vi "getCharactersv2.vi"(0 "ocr in":refnum<class "ocr.lvclass">, 5 "noofImgs":i32=1, 11 "error in (no error)":errorcluster) -> (4 "ocr out":refnum<class "ocr.lvclass">, 6 "succ":i32, 8 "OCRResultB":T1[](array[typedef]), 15 "error out":errorcluster)   [LabVIEW 2025, in "adsOCR.lvlib" / "ocr.lvclass"]
uses:
  ocr.lvclass
  ocrImageResult.ctl
  ocrDetection.ctl
  ocr.lvclass/ocr.ctl
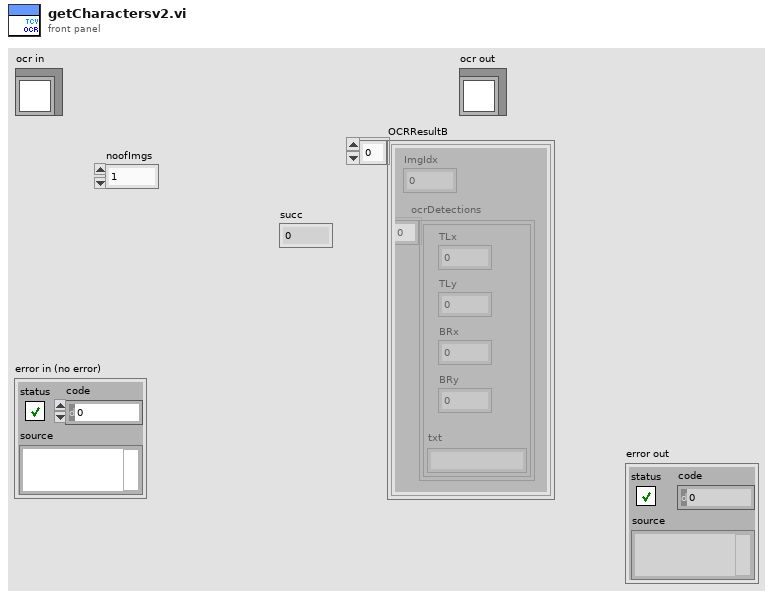
[diagram p1: front panel]
types:
  T1 = typedef "adsOCR.lvlib/ocr.lvclass/ocrImageResult.ctl" = cluster{"ImgIdx":i16, "ocrDetections":T2[]}
  T2 = typedef "adsOCR.lvlib/ocr.lvclass/ocrDetection.ctl" = cluster{"TLx":i32, "TLy":i32, "BRx":i32, "BRy":i32, "txt":string}
  T3 = typedef "adsOCR.lvlib/ocr.lvclass/TextDecRecResult2L.ctl" = cluster{"imgIdx":i32, "TLx":i32, "TLy":i32, "BRx":i32, "BRy":i32, "angle":sgl, "txtLen":i32}
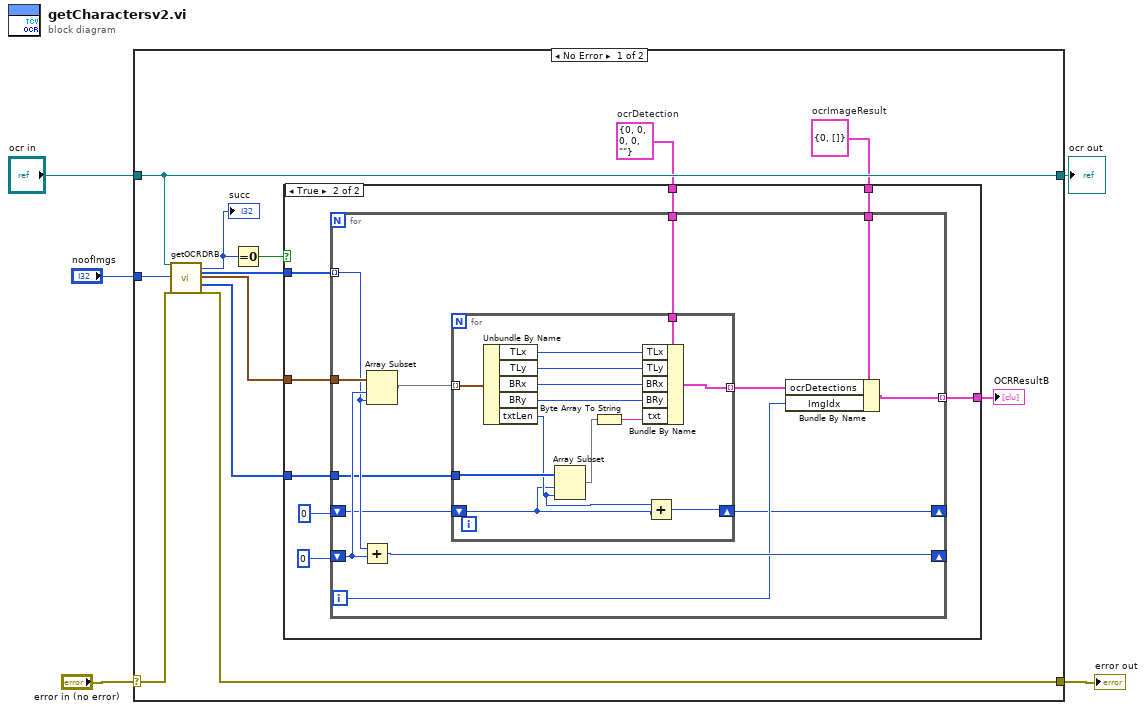
[diagram p0: block diagram]
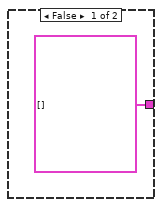
[diagram p2: hidden frame]
diagram:
  n1 = case shown="No Error" "error in (no error)" {
    selector: "error in (no error)" -> [w7 w54]
    tunnel: [w6 w54] -> w4
    tunnel: [w17 w53] -> w2
    tunnel: "ocr in" -> [w17 w53]
    tunnel: "noofImgs" -> [w16 _]
    frame No Error {
      w11 = T2 {"TLx"=0, "TLy"=0, "BRx"=0, "BRy"=0, "txt"=""}  # ocrDetection
      w9 = T1 {"ImgIdx"=0, "ocrDetections"=[]}  # ocrImageResult
      n2 = call-dynamic "getOCRDRB.vi"("ocr in"=w17, "noofImgs"=w16, "error in (no error)"=w7) -> ("succ"=w14:i32, "countsPerImg"=w13:i32[], "TextDecRecResult2L"=w12:T3[], "Chars"=w10:u8[], "error out"=w6:errorcluster)  [unwired: 18 in, 2 out]
      "succ" <- w14
      n3 = Equal To 0?(x=w14) -> (x = 0?=w15:bool)
      n4 = case shown="True" w15 {
        tunnel: w13 -> [_ w26]
        tunnel: w12 -> [_ w25]
        tunnel: w11 -> [_ w23]
        tunnel: w10 -> [_ w22]
        tunnel: w9 -> [_ w21]
        tunnel: [T1[] [] w20] -> w8
        frame False {
        }
        frame True {
          n5 = for {
            shift-right: [w38] -> _
            shift-left: 0 -> [w37]
            tunnel: w26 -> [w36] mode=indexing
            tunnel: w25 -> [w39]
            tunnel: w23 -> [w34]
            tunnel: w22 -> [w33]
            tunnel: w21 -> [w32]
            tunnel: [w29] -> w20 mode=indexing
            shift-right: [w27] -> _
            shift-left: 0 -> [w28]
            i -> [w31]
            n6 = Add(x=w36, y=w37) -> (x+y=w38:i32)
            n7 = Array Subset(array=w39, index=w37, length=w36) -> (w35:T3[])
            n8 = for {
              tunnel: w35 -> [w52] mode=indexing
              tunnel: w34 -> [w51]
              tunnel: w33 -> [w46]
              tunnel: [w43] -> w30 mode=indexing
              shift-right: [w42] -> w27
              shift-left: w28 -> [w40]
              n9 = Unbundle By Name(w52) -> ("TLx"=w50:i32, "TLy"=w49:i32, "BRx"=w48:i32, "BRy"=w47:i32, "txtLen"=w41:i32)
              n10 = Array Subset(array=w46, index=w40, length=w41) -> (w45:u8[])
              n11 = Byte Array To String(unsigned byte array=w45) -> (string=w44:string)
              n12 = Bundle By Name(cluster=w51, "TLx"=w50, "TLy"=w49, "BRx"=w48, "BRy"=w47, "txt"=w44) -> (w43:T2)
              n13 = Add(x=w41, y=w40) -> (x+y=w42:i32)
            }
            n14 = Bundle By Name(cluster=w32, "ocrDetections"=w30, "ImgIdx"=w31) -> (w29:T1)
          }
        }
      }
      "OCRResultB" <- w8
    }
    frame Error {
    }
  }
  "error out" <- w4
  "ocr out" <- w2
